vi "Add Readme Resource.vi"(8 "error in":errorcluster, 10 "readme path":path, 11 "server id":i32) -> (0 "error out":errorcluster, 3 "server id out":i32)   [LabVIEW 2020]
doc: "Registers a readme file as an MCP resource, so that a client can read how the example works.\n\nBy default it is the readme.md of the Datalogger example. That path is built at run time: readme.md lies in the folder above the folder of this VI.\n\nA caller can register a different file with readme path. If readme path is empty or not a valid path, the default readme.md is used.\n\nName and uri of the resource come from the file name (Add Resource (File).vi): readme.md gives the name readme and the uri labview://readme, another file gives its own name."
uses:
  src/MCP Server/MCP Server.lvlib
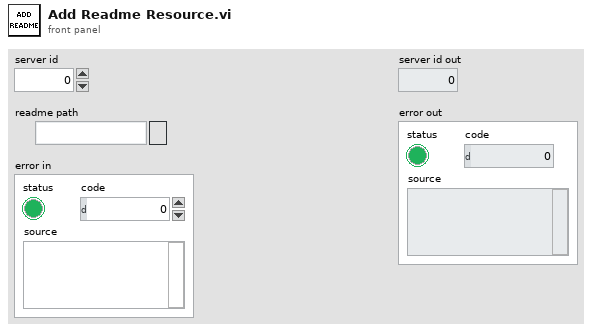
[diagram p1: front panel]
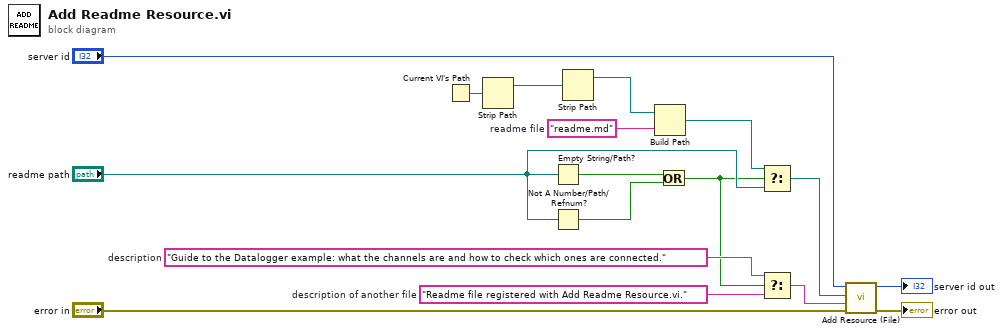
[diagram p0: block diagram]
diagram:
  w7 = "Readme file registered with Add Readme Resource.vi."  # description of another file
  w9 = "Guide to the Datalogger example: what the channels are and how to check which ones are connected."  # description
  w14 = "readme.md"  # readme file
  n1 = Current VI's Path() -> (path=w17:path)
  n2 = Strip Path(path=w17) -> (stripped path=w16:path)  [unwired: 1 out]
  n3 = Empty String/Path?(string/path="readme path") -> (empty?=w13:bool)
  n4 = Not A Number/Path/Refnum?(number/path/refnum="readme path") -> (NaN/Path/Refnum?=w12:bool)
  n5 = Strip Path(path=w16) -> (stripped path=w15:path)  [unwired: 1 out]
  n6 = Build Path(base path=w15, name or relative path=w14) -> (appended path=w11:path)
  n7 = Or(x=w13, y=w12) -> (x .or. y?=w8:bool)
  n8 = Select(t=w11, s=w8, f="readme path") -> (s? t:f=w5:path)
  n9 = Select(t=w9, s=w8, f=w7) -> (s? t:f=w4:string)
  n10 = call "Add Resource (File).vi"("error in (no error)"="error in", "description"=w4, "file path"=w5, "server id"="server id") -> ("error out"=→"error out":errorcluster, "server id out"=→"server id out":i32)  [unwired: 6 in]
